vi "test_PhotonPoseEstimator_lowestAmbiguity.vi"(8 "error in (no error)":errorcluster) -> (0 "error out":errorcluster, 3 "Test Passed":bool)   [LabVIEW 2019]
uses:
  <vilib>/Rock Robotics/WPI/ThirdParty/PhotonVisionLib/TypeDef/PhotonEstimatedRobotPoseType.ctl
  <vilib>/Rock Robotics/WPI/ThirdParty/JAS_Junk/TrajLib/TypeDef/POSE3D.ctl
  <vilib>/Rock Robotics/WPI/ThirdParty/JAS_Junk/TrajLib/TypeDef/TRANSLATION3D.ctl
  <vilib>/Rock Robotics/WPI/ThirdParty/JAS_Junk/TrajLib/TypeDef/ROTATION3D.ctl
  <vilib>/Rock Robotics/WPI/ThirdParty/JAS_Junk/TrajLib/TypeDef/QUATERNION.ctl
  <vilib>/Rock Robotics/WPI/ThirdParty/PhotonVisionLib/TypeDef/PhotonTrackedTargetType.ctl
  <vilib>/Rock Robotics/WPI/ThirdParty/PhotonVisionLib/TypeDef/TargetCornerType.ctl
  <vilib>/Rock Robotics/WPI/ThirdParty/JAS_Junk/TrajLib/TypeDef/TRANSFORM3D.ctl
  <vilib>/Rock Robotics/WPI/ThirdParty/PhotonVisionLib/Enum/PhotonPoseStrategy_ENUM.ctl
  <vilib>/Rock Robotics/WPI/ThirdParty/JAS_Junk/TrajLib/VI/Translation3d_Create_Default.vi
  <vilib>/Rock Robotics/WPI/ThirdParty/JAS_Junk/TrajLib/VI/Rotation3d_Create_Default.vi
  <vilib>/Rock Robotics/WPI/ThirdParty/PhotonVisionLib/SubVI/PhotonTargetModel_New_AprilTag36H11.vi
  <vilib>/Rock Robotics/WPI/ThirdParty/JAS_Junk/TrajLib/VI/TimeInterpRotation2d_New.vi
  <vilib>/Rock Robotics/WPI/ThirdParty/JAS_Junk/TrajLib/VI/Quaternion_New.vi
  <vilib>/Rock Robotics/WPI/ThirdParty/PhotonVisionLib/SubVI/PhotonPoseEstimator_Update_All.vi
  <vilib>/Rock Robotics/WPI/ThirdParty/JAS_Junk/TrajLib/VI/Quaternion_New_Default.vi
  <vilib>/Rock Robotics/WPI/ThirdParty/PhotonVisionLib/SubVI/PhotonTargetModel_New_RectPlanar.vi
  <vilib>/Rock Robotics/WPI/ThirdParty/JAS_Junk/TrajLib/Conv_Inches_Meters.vi
  <vilib>/Rock Robotics/WPI/ThirdParty/PhotonVisionLib/SubVI/PhotonPoseEstimator_SetLastPose.vi
  <vilib>/Rock Robotics/WPI/ThirdParty/PhotonVisionLib/SubVI/PhotonPoseEstimator_GetEmptyPose.vi
  <vilib>/Rock Robotics/WPI/ThirdParty/PhotonVisionLib/SubVI/PhotonPoseEstimator_EstimateLowestAmbiguityPose.vi
  <vilib>/Rock Robotics/WPI/ThirdParty/PhotonVisionLib/SubVI/PhotonPoseEstimator_EstimateClosestToCameraHeightPose.vi
  <vilib>/Rock Robotics/WPI/ThirdParty/PhotonVisionLib/SubVI/PhotonPoseEstimator_EstimateClosestToReferencePose.vi
  <vilib>/Rock Robotics/WPI/ThirdParty/PhotonVisionLib/SubVI/PhotonPoseEstimator_GetReferencePose.vi
  <vilib>/Rock Robotics/WPI/ThirdParty/PhotonVisionLib/SubVI/PhotonPoseEstimator_GetLastPose.vi
  <vilib>/Rock Robotics/WPI/ThirdParty/PhotonVisionLib/SubVI/PhotonPoseEstimator_SetReferencePose.vi
  <vilib>/Rock Robotics/WPI/ThirdParty/PhotonVisionLib/SubVI/PhotonPoseEstimator_EstimateClosestToLastPose.vi
  <vilib>/Rock Robotics/WPI/ThirdParty/PhotonVisionLib/SubVI/PhotonPoseEstimator_EstimateAverageBestTargetsPose.vi
  <vilib>/Rock Robotics/WPI/ThirdParty/PhotonVisionLib/SubVI/PhotonPoseEstimator_EstimateMultiTagOnCoprocPose.vi
  <vilib>/Rock Robotics/WPI/ThirdParty/PhotonVisionLib/SubVI/PhotonPoseEstimator_EstimatePnpDistanceTrigSolvePose.vi
  <vilib>/Rock Robotics/WPI/ThirdParty/PhotonVisionLib/SubVI/PhotonPoseEstimator_Strategy_constrainedPnpStrategy.vi
  <vilib>/Rock Robotics/WPI/ThirdParty/PhotonVisionLib/SubVI/PhotonPipelineResult_GetTimeStampSecs.vi
  <vilib>/Rock Robotics/WPI/ThirdParty/PhotonVisionLib/SubVI/PhotonTargetModel_New.vi
  <vilib>/Rock Robotics/WPI/ThirdParty/JAS_Junk/TrajLib/VI/Rotation3d_Create_AxisAngle.vi
  <vilib>/Rock Robotics/WPI/ThirdParty/JAS_Junk/TrajLib/VI/Pose3d_New.vi
  <vilib>/Rock Robotics/WPI/ThirdParty/PhotonVisionLib/SubVI/PhotonPipelineResult_HasTargets.vi
  <vilib>/Rock Robotics/WPI/ThirdParty/PhotonVisionLib/SubVI/PhotonPipelineResult_GetTargets.vi
  <vilib>/Rock Robotics/WPI/ThirdParty/PhotonVisionLib/SubVI/PhotonTrackedTarget_GetPoseAmbiguity.vi
  <vilib>/Rock Robotics/WPI/ThirdParty/PhotonVisionLib/SubVI/PhotonTrackedTarget_GetFiducialId.vi
  <vilib>/Rock Robotics/WPI/ThirdParty/PhotonVisionLib/SubVI/PhotonPoseEstimator_GetFieldTags.vi
  <vilib>/Rock Robotics/WPI/ThirdParty/JAS_Junk/TrajLib/VI/AprilTagFieldLayout_GetTagPose.vi
  <vilib>/Rock Robotics/WPI/ThirdParty/JAS_Junk/TrajLib/VI/Pose3d_TransformBy.vi
  <vilib>/Rock Robotics/WPI/ThirdParty/PhotonVisionLib/SubVI/PhotonTrackedTarget_GetBestCameraToTarget.vi
  <vilib>/Rock Robotics/WPI/ThirdParty/JAS_Junk/TrajLib/VI/Transform3d_Inverse.vi
  <vilib>/Rock Robotics/WPI/ThirdParty/PhotonVisionLib/SubVI/PhotonPoseEstimator_GetRobotToCameraTransform.vi
  <vilib>/Rock Robotics/WPI/ThirdParty/PhotonVisionLib/SubVI/PhotonPoseEstimator_GetHighestAmbiguity.vi
  <vilib>/Rock Robotics/WPI/ThirdParty/PhotonVisionLib/SubVI/PhotonEstimatedRobotPose_New.vi
  <vilib>/Rock Robotics/WPI/ThirdParty/PhotonVisionLib/SubVI/PhotonPoseEstimator_Strategy_closestToCameraHeight_calc.vi
  <vilib>/Rock Robotics/WPI/ThirdParty/PhotonVisionLib/SubVI/PhotonTrackedTarget_GetAltCameraToTarget.vi
  <vilib>/Rock Robotics/WPI/ThirdParty/PhotonVisionLib/SubVI/PhotonPoseEstimator_Strategy_closestToReferencePose_calc.vi
  <vilib>/Rock Robotics/WPI/ThirdParty/PhotonVisionLib/SubVI/PhotonPoseEstimator_Strategy_averageBestTargets_calc.vi
  <vilib>/Rock Robotics/WPI/ThirdParty/JAS_Junk/TrajLib/VI/Rotation3d_Plus.vi
  <vilib>/Rock Robotics/WPI/ThirdParty/JAS_Junk/TrajLib/VI/Translation3d_Plus.vi
  <vilib>/Rock Robotics/WPI/ThirdParty/JAS_Junk/TrajLib/VI/Translation3d_Times.vi
  <vilib>/Rock Robotics/WPI/ThirdParty/JAS_Junk/TrajLib/VI/Rotation3d_Times.vi
  <vilib>/Rock Robotics/WPI/ThirdParty/JAS_Junk/TrajLib/VI/Pose3d_New_Trans3dRot3d.vi
  <vilib>/Rock Robotics/WPI/ThirdParty/JAS_Junk/TrajLib/VI/Pose3d_New_Default.vi
  <vilib>/Rock Robotics/WPI/ThirdParty/JAS_Junk/TrajLib/VI/Pose3d_Plus.vi
  <vilib>/Rock Robotics/WPI/ThirdParty/JAS_Junk/TrajLib/VI/Pose3d_RelativeTo.vi
  <vilib>/Rock Robotics/WPI/ThirdParty/JAS_Junk/TrajLib/VI/AprilTagFieldLayout_GetOriginPosition.vi
  <vilib>/Rock Robotics/WPI/ThirdParty/PhotonVisionLib/SubVI/PhotonPipelineResult_GetMultiTagResult.vi
  <vilib>/Rock Robotics/WPI/ThirdParty/PhotonVisionLib/SubVI/PhotonPipelineResult_GetBestTarget.vi
  <vilib>/Rock Robotics/WPI/ThirdParty/PhotonVisionLib/SubVI/PhotonTrackedTarget_GetPitch.vi
  <vilib>/Rock Robotics/WPI/ThirdParty/PhotonVisionLib/SubVI/PhotonTrackedTarget_GetYaw.vi
  <vilib>/Rock Robotics/WPI/ThirdParty/JAS_Junk/TrajLib/Units_DegreesToRadians.vi
  <vilib>/Rock Robotics/WPI/ThirdParty/JAS_Junk/TrajLib/VI/Transform3d_GetTranslation3d.vi
  <vilib>/Rock Robotics/WPI/ThirdParty/JAS_Junk/TrajLib/VI/Translation3d_GetNorm.vi
  <vilib>/Rock Robotics/WPI/ThirdParty/JAS_Junk/TrajLib/VI/Translation3d_Create_DistAng.vi
  <vilib>/Rock Robotics/WPI/ThirdParty/JAS_Junk/TrajLib/VI/Translation3d_RotateBy.vi
  <vilib>/Rock Robotics/WPI/ThirdParty/JAS_Junk/TrajLib/VI/Translation3d_ToTranslation2d.vi
  <vilib>/Rock Robotics/WPI/ThirdParty/JAS_Junk/TrajLib/Translation2d_RotateBy.vi
  <vilib>/Rock Robotics/WPI/ThirdParty/JAS_Junk/TrajLib/VI/Transform3d_GetRotation3d.vi
  <vilib>/Rock Robotics/WPI/ThirdParty/JAS_Junk/TrajLib/VI/Pose3d_ToPose2d.vi
  <vilib>/Rock Robotics/WPI/ThirdParty/JAS_Junk/TrajLib/Pose2d_getTranslation.vi
  <vilib>/Rock Robotics/WPI/ThirdParty/JAS_Junk/TrajLib/Translation2d_Plus.vi
  <vilib>/Rock Robotics/WPI/ThirdParty/JAS_Junk/TrajLib/Translation2d_UnaryMinus.vi
  <vilib>/Rock Robotics/WPI/ThirdParty/JAS_Junk/TrajLib/Pose2d_New_TRRO.vi
  <vilib>/Rock Robotics/WPI/ThirdParty/JAS_Junk/TrajLib/VI/Pose3d_New_Pose2d.vi
  <vilib>/Rock Robotics/WPI/ThirdParty/JAS_Junk/TrajLib/VI/TimeInterpRotation2d_GetSample.vi
  <vilib>/Rock Robotics/WPI/ThirdParty/PhotonVisionLib/SubVI/PhotonPoseEstimator_GetHeadingBuffer.vi
  <vilib>/Rock Robotics/WPI/ThirdParty/JAS_Junk/TrajLib/VI/Vector_Norm.vi
  <vilib>/Rock Robotics/WPI/ThirdParty/JAS_Junk/TrajLib/VecBuilder_ArrayBy1Fill.vi
  <vilib>/Rock Robotics/WPI/ThirdParty/JAS_Junk/TrajLib/VI/AprilTag_GetAll.vi
  <vilib>/Rock Robotics/WPI/ThirdParty/JAS_Junk/TrajLib/VI/Pose3d_getTranslation3d.vi
  <vilib>/Rock Robotics/WPI/ThirdParty/JAS_Junk/TrajLib/VI/Pose3d_getRotation3d.vi
  <vilib>/Rock Robotics/WPI/ThirdParty/JAS_Junk/TrajLib/VI/Rotation3d_ToRotation2d.vi
  <vilib>/Rock Robotics/WPI/ThirdParty/JAS_Junk/TrajLib/Transform2d_Create_TransRot.vi
  <vilib>/Rock Robotics/WPI/ThirdParty/JAS_Junk/TrajLib/VI/Rotation3d_UnaryMinus.vi
  <vilib>/Rock Robotics/WPI/ThirdParty/JAS_Junk/TrajLib/VI/Translation3d_UnaryMinus.vi
  <vilib>/Rock Robotics/WPI/ThirdParty/JAS_Junk/TrajLib/VI/Transform3d_GetXYZ.vi
  <vilib>/Rock Robotics/WPI/ThirdParty/JAS_Junk/TrajLib/VI/Pose3d_getXYZ.vi
  <vilib>/Rock Robotics/WPI/ThirdParty/PhotonVisionLib/SubVI/PhotonPoseEstimator_CalcDifference.vi
  <vilib>/Rock Robotics/WPI/ThirdParty/JAS_Junk/TrajLib/VI/Rotation3d_RotateBy.vi
  <vilib>/Rock Robotics/WPI/ThirdParty/JAS_Junk/TrajLib/VI/Translation3d_GetXYZ.vi
  <vilib>/Rock Robotics/WPI/ThirdParty/JAS_Junk/TrajLib/VI/Rotation3d_GetQuaterion.vi
  <vilib>/Rock Robotics/WPI/ThirdParty/JAS_Junk/TrajLib/VI/Quaternion_Get_Vect.vi
  <vilib>/Rock Robotics/WPI/ThirdParty/JAS_Junk/TrajLib/VI/Quaternion_Get_W.vi
  <vilib>/Rock Robotics/WPI/ThirdParty/JAS_Junk/TrajLib/VI/Transform3d_Create_Pose3dPose3d.vi
  <vilib>/Rock Robotics/WPI/ThirdParty/JAS_Junk/TrajLib/Conv_Deg_Radians.vi
  <vilib>/Rock Robotics/WPI/ThirdParty/JAS_Junk/TrajLib/VI/Quaternion_Times.vi
  <vilib>/Rock Robotics/WPI/ThirdParty/JAS_Junk/TrajLib/VI/Quaternion_Inverse.vi
  <vilib>/Rock Robotics/WPI/ThirdParty/JAS_Junk/TrajLib/VI/Quaternion_Get_All.vi
  <vilib>/Rock Robotics/WPI/ThirdParty/JAS_Junk/TrajLib/Translation2d_Create.vi
  <vilib>/Rock Robotics/WPI/ThirdParty/JAS_Junk/TrajLib/Pose2d_getXYAngle.vi
  <vilib>/Rock Robotics/WPI/ThirdParty/JAS_Junk/TrajLib/Rotation2d_Interpolate.vi
  <vilib>/Rock Robotics/WPI/ThirdParty/JAS_Junk/TrajLib/MatBuilder_Create.vi
  <vilib>/Rock Robotics/WPI/ThirdParty/JAS_Junk/TrajLib/Rotation2d_CreateAngle.vi
  <vilib>/Rock Robotics/WPI/ThirdParty/JAS_Junk/TrajLib/VI/Rotation3d_GetXYZ.vi
  <vilib>/Rock Robotics/WPI/ThirdParty/JAS_Junk/TrajLib/VI/Rotation3d_Create_Quaternion.vi
  <vilib>/Rock Robotics/WPI/ThirdParty/JAS_Junk/TrajLib/VI/Translation3d_GetDistance.vi
  <vilib>/Rock Robotics/WPI/ThirdParty/JAS_Junk/TrajLib/VI/Translation3d_Minus.vi
  <vilib>/Rock Robotics/WPI/ThirdParty/JAS_Junk/TrajLib/VI/Rotation3d_Minus.vi
  <vilib>/Rock Robotics/WPI/ThirdParty/JAS_Junk/TrajLib/Rotation2d_Plus.vi
  <vilib>/Rock Robotics/WPI/ThirdParty/JAS_Junk/TrajLib/Rotation2d_Minus.vi
  <vilib>/Rock Robotics/WPI/ThirdParty/JAS_Junk/TrajLib/MathUtil_Clamp.vi
  <vilib>/Rock Robotics/WPI/ThirdParty/JAS_Junk/TrajLib/Rotation2d_Times.vi
  <vilib>/Rock Robotics/WPI/ThirdParty/JAS_Junk/TrajLib/VI/Quaternion_Normalize.vi
  <vilib>/Rock Robotics/WPI/ThirdParty/JAS_Junk/TrajLib/Rotation2d_RotateBy.vi
  <vilib>/Rock Robotics/WPI/ThirdParty/JAS_Junk/TrajLib/Rotation2d_UnaryMinus.vi
  <vilib>/Rock Robotics/WPI/ThirdParty/JAS_Junk/TrajLib/Rotation2d_CreateXY.vi
  <vilib>/Rock Robotics/WPI/ThirdParty/JAS_Junk/TrajLib/Util_CalcDist.vi
  <vilib>/Rock Robotics/WPI/ThirdParty/PhotonVisionLib/SubVI/PhotonVision_Globals.vi
  <vilib>/gmath/interp.llb/Search Ordered Table.vi
  <vilib>/Rock Robotics/WPI/ThirdParty/JAS_Junk/TrajLib/Trajectory_Library.lvlib
  <vilib>/Rock Robotics/WPI/ThirdParty/PhotonVisionLib/PhotonVisionLib.lvlib
panel:
  out "Test 2 Passed":bool
  out "Test 1 Passed":bool
  out "Pos Found":bool
  out "PhotonEstimatedRobotPose":T1={"EstimatedPose"={"Translation3d"={"X"=0.0, "Y"=0.0, "Z"=0.0}, "Rotation3d"={"Q_quaternion"={"R"=1.0, "V"=[0.0, 0.0, 0.0]}}}, "TimeStamp_Seconds"=0.0, "targetsUsed"=[], "Strategy"=enum."LOWEST_AMBIGUITY"} {"targetsUsed"."AltCameraToTarget"."TRANSLATION3D"."Z" format="%14.3f"; "targetsUsed"."AltCameraToTarget"."TRANSLATION3D"."Y" format="%14.3f"; "targetsUsed"."AltCameraToTarget"."TRANSLATION3D"."X" format="%14.3f"; "targetsUsed"."BestCameraToTarget"."TRANSLATION3D"."Z" format="%14.3f"; "targetsUsed"."BestCameraToTarget"."TRANSLATION3D"."Y" format="%14.3f"; "targetsUsed"."BestCameraToTarget"."TRANSLATION3D"."X" format="%14.3f"; "EstimatedPose"."Translation3d"."Z" format="%14.3f"; "EstimatedPose"."Translation3d"."Y" format="%14.3f"; "EstimatedPose"."Translation3d"."X" format="%14.3f"}
  out "Test 0 Passed":bool
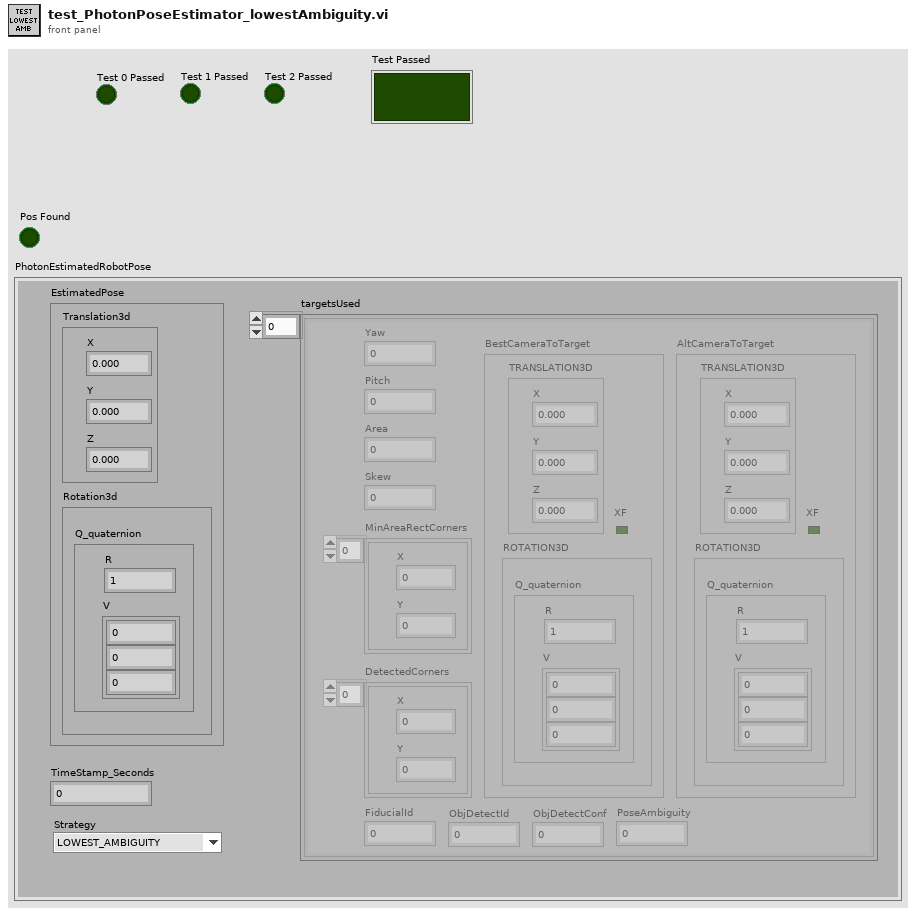
[diagram p1: front panel]
types:
  T1 = typedef "PhotonVisionLib.lvlib/PhotonEstimatedRobotPoseType.ctl" = cluster{"EstimatedPose":T2, "TimeStamp_Seconds":dbl, "targetsUsed":T6[], "Strategy":T9}
  T2 = typedef "Trajectory_Library.lvlib/POSE3D.ctl" = cluster{"Translation3d":T3, "Rotation3d":T4}
  T3 = typedef "Trajectory_Library.lvlib/TRANSLATION3D.ctl" = cluster{"X":dbl, "Y":dbl, "Z":dbl}
  T4 = typedef "Trajectory_Library.lvlib/ROTATION3D.ctl" = cluster{"Q_quaternion":T5}
  T5 = typedef "Trajectory_Library.lvlib/QUATERNION.ctl" = cluster{"R":dbl, "V":dbl[]}
  T6 = typedef "PhotonVisionLib.lvlib/PhotonTrackedTargetType.ctl" = cluster{"Yaw":dbl, "Pitch":dbl, "Area":dbl, "Skew":dbl, "MinAreaRectCorners":T7[], "BestCameraToTarget":T8, "FiducialId":i32, "AltCameraToTarget":T8, "PoseAmbiguity":dbl, "DetectedCorners":T7[], "ObjDetectId":i32, "ObjDetectConf":sgl}
  T7 = typedef "PhotonVisionLib.lvlib/TargetCornerType.ctl" = cluster{"X":dbl, "Y":dbl}
  T8 = typedef "Trajectory_Library.lvlib/TRANSFORM3D.ctl" = cluster{"TRANSLATION3D":T3, "ROTATION3D":T4, "XF":bool}
  T9 = typedef "PhotonVisionLib.lvlib/PhotonPoseStrategy_ENUM.ctl" = enum16{"LOWEST_AMBIGUITY", "CLOSEST_TO_CAMERA_HEIGHT", "CLOSEST_TO_REFERENCE_POSE", "CLOSEST_TO_LAST_POSE", "AVERAGE_BEST_TARGETS", "MULTI_TAG_PNP_ON_COPROCESSOR", "MULTI_TAG_PNP_ON_RIO", "PNP_DISTANCE_TRIG_SOLVE", "CONSTRAINED_SOLVEPNP"}
  T10 = typedef "Trajectory_Library.lvlib/AprilTagFieldLayout.ctl" = cluster{"AprilTagMap":map{i32, T11}, "FieldLength":dbl, "FieldWidth":dbl, "OriginPosition ":T12, "OriginPose3d":T2}
  T11 = typedef "Trajectory_Library.lvlib/AprilTag.ctl" = cluster{"ID":i32, "POSE3D":T2}
  T12 = typedef "Trajectory_Library.lvlib/AprilTagFieldLayoutOrignPosition_ENUM.ctl" = enum16{"kBlueAllianceWallRightSide,", "kRedAllianceWallRightSide,"}
  T13 = typedef "PhotonVisionLib.lvlib/PhotonPipelineMetadataType.ctl" = cluster{"CaptureTimestampMicros":i64, "PublishTimestampMicros":i64, "SequenceID":i64, "TimeSinceLastPong":i64}
  T14 = typedef "PhotonVisionLib.lvlib/PhotonPipelineResultType.ctl" = cluster{"Targets":T6[], "PhotonMultiTargetPNPResult":T15, "PhotonPipelineMetadata":T13}
  T15 = typedef "PhotonVisionLib.lvlib/PhotonMultiTargetPNPResultType.ctl" = cluster{"PhotonPNPResult":T16, "FiducialIDsUsed":i16[]}
  T16 = typedef "PhotonVisionLib.lvlib/PhotonPNPResultType.ctl" = cluster{"IsPresent":bool, "bestReprojErr":dbl, "altReprojErr":dbl, "ambiguity":dbl, "Best":T8, "Alt":T8}
  T17 = typedef "PhotonVisionLib.lvlib/PhotonPoseEstimatorType.ctl" = cluster{"LastPose":T2, "ReferencePose":T2, "FieldTags":T10, "PrimaryStratety":T9, "Camera":string, "RobotToCamera":T8, "ReportedErrors":dbl[], "HighestAmbiguity":dbl, "MultiTagFallbackStrategy":T9, "PoseCacheTimeoutSec":dbl, "PhotonTargetModel":T18, "BaseNTName":string}
  T18 = typedef "PhotonVisionLib.lvlib/PhotonTargetModel.ctl" = cluster{"Vertices":T3[], "IsPlaner":bool, "IsSpherical":bool}
  T19 = typedef "PhotonVisionLib.lvlib/PhotonPoseEstimator_Configuration.ctl" = cluster{"Primary Strategy":T9, "Camera":string, "Initial Pose":T2, "HighestAmbiguity":dbl, "RobotToCamera":T8, "FallBack Strategy":T9, "BaseNTName":string}
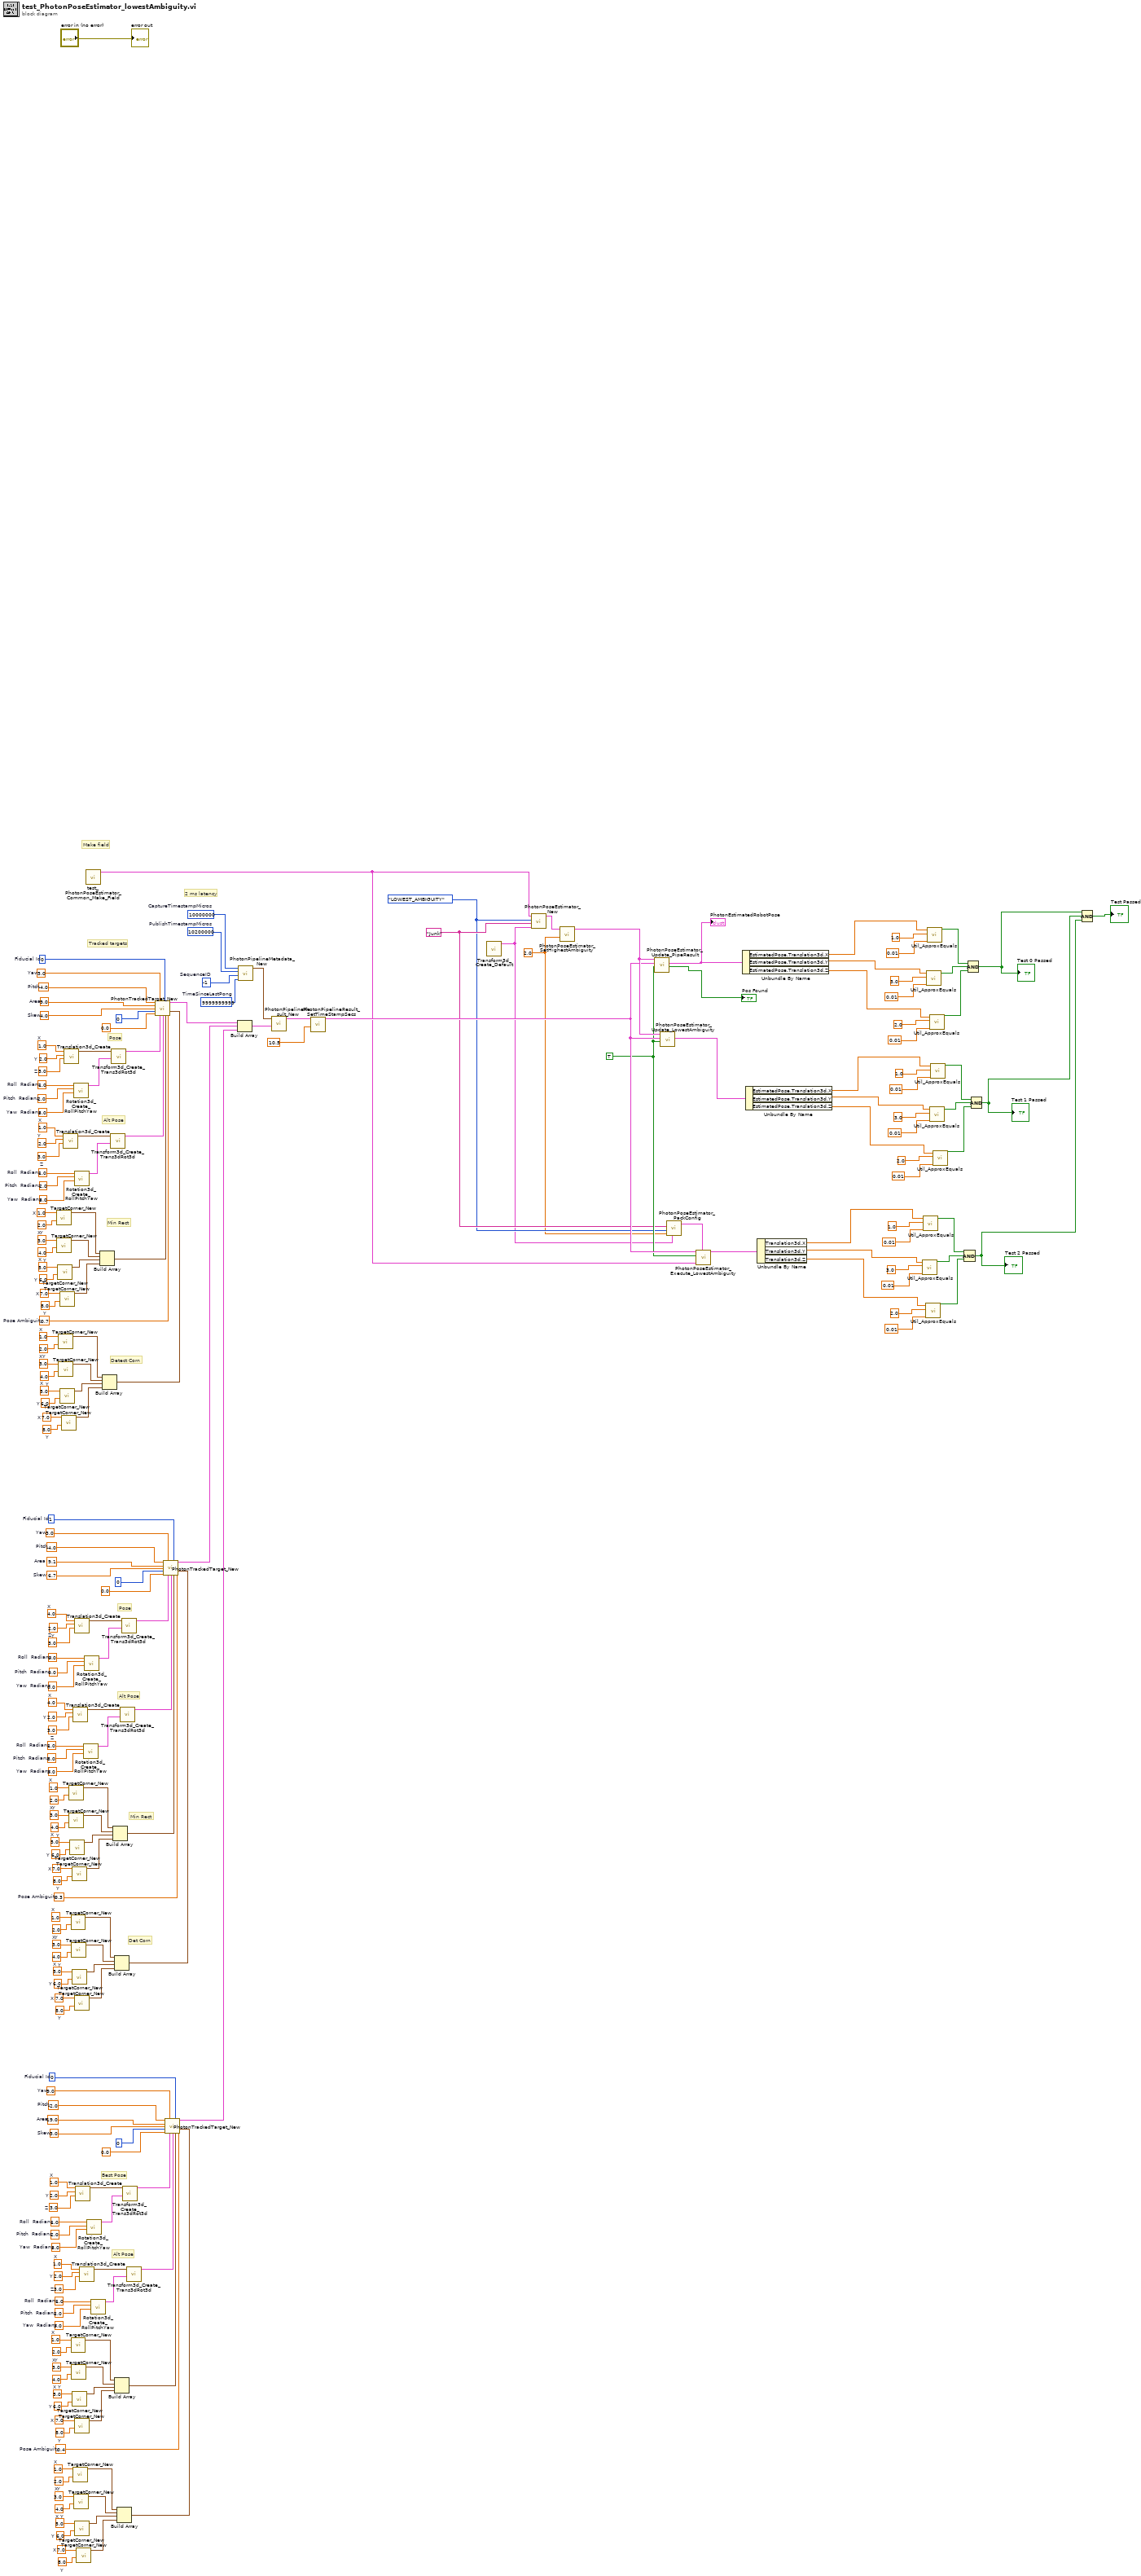
[diagram p0: block diagram]
diagram:
  w2 = 2.0 ("HighestAmbiguity")
  w46 = i64 10000000  # CaptureTimestampMicros
  w47 = i64 10200000  # PublishTimestampMicros
  w48 = i64 -1  # SequenceID
  w49 = i64 9999999999  # TimeSinceLastPong
  w20 = TRUE ("Has Results")
  w4 = "Junk" ("Camera")
  w3 = PhotonPoseStrategy_ENUM."LOWEST_AMBIGUITY" ("Strategy")
  w73 = 1.0  # Roll  Radians
  w72 = 2.0  # Pitch  Radians
  w71 = 3.0  # Yaw  Radians
  w76 = 3.0  # Z
  w75 = 1.0  # X
  w74 = 2.0  # Y
  w81 = 1.0  # Roll  Radians
  w80 = 2.0  # Pitch  Radians
  w79 = 3.0  # Yaw  Radians
  w84 = 3.0  # Z
  w83 = 1.0  # X
  w82 = 2.0  # Y
  w91 = 7.0  # X
  w92 = 8.0  # Y
  w93 = 5.0  # X
  w94 = 6.0  # Y
  w95 = 3.0  # X
  w96 = 4.0  # Y
  w97 = 1.0  # X
  w98 = 2.0  # Y
  w103 = 7.0  # X
  w104 = 8.0  # Y
  w105 = 5.0  # X
  w106 = 6.0  # Y
  w107 = 3.0  # X
  w108 = 4.0  # Y
  w109 = 1.0  # X
  w110 = 2.0  # Y
  w111 = -2.0  # Pitch
  w112 = 19.0  # Area
  w113 = 3.0  # Skew
  w114 = 0  # Fiducial Id
  w115 = 0.4  # Pose Ambiguity
  w116 = 9.0  # Yaw
  w123 = 0.0  # Roll  Radians
  w122 = 0.0  # Pitch  Radians
  w121 = 0.0  # Yaw  Radians
  w126 = 3.0  # Z
  w125 = 4.0  # X
  w124 = 2.0  # Y
  w131 = 1.0  # Roll  Radians
  w130 = 5.0  # Pitch  Radians
  w129 = 3.0  # Yaw  Radians
  w134 = 3.0  # Z
  w133 = 4.0  # X
  w132 = 2.0  # Y
  w141 = 7.0  # X
  w142 = 8.0  # Y
  w143 = 5.0  # X
  w144 = 6.0  # Y
  w145 = 3.0  # X
  w146 = 4.0  # Y
  w147 = 1.0  # X
  w148 = 2.0  # Y
  w153 = 7.0  # X
  w154 = 8.0  # Y
  w155 = 5.0  # X
  w156 = 6.0  # Y
  w157 = 3.0  # X
  w158 = 4.0  # Y
  w159 = 1.0  # X
  w160 = 2.0  # Y
  w161 = -4.0  # Pitch
  w162 = 9.1  # Area
  w163 = 6.7  # Skew
  w164 = 1  # Fiducial Id
  w165 = 0.3  # Pose Ambiguity
  w166 = 3.0  # Yaw
  w173 = 1.0  # Roll  Radians
  w172 = 2.0  # Pitch  Radians
  w171 = 3.0  # Yaw  Radians
  w176 = 3.0  # Z
  w175 = 1.0  # X
  w174 = 2.0  # Y
  w181 = 1.0  # Roll  Radians
  w180 = 2.0  # Pitch  Radians
  w179 = 3.0  # Yaw  Radians
  w184 = 3.0  # Z
  w183 = 1.0  # X
  w182 = 2.0  # Y
  w191 = 7.0  # X
  w192 = 8.0  # Y
  w193 = 5.0  # X
  w194 = 6.0  # Y
  w195 = 3.0  # X
  w196 = 4.0  # Y
  w197 = 1.0  # X
  w198 = 2.0  # Y
  w203 = 7.0  # X
  w204 = 8.0  # Y
  w205 = 5.0  # X
  w206 = 6.0  # Y
  w207 = 3.0  # X
  w208 = 4.0  # Y
  w209 = 1.0  # X
  w210 = 2.0  # Y
  w211 = -4.0  # Pitch
  w212 = 9.0  # Area
  w213 = 4.0  # Skew
  w214 = 0  # Fiducial Id
  w215 = 0.7  # Pose Ambiguity
  w216 = 3.0  # Yaw
  # "2 ms latency"
  # "Det Corn"
  # "Min Rect"
  # "Pose"
  # "Detect Corn"
  # "Min Rect"
  # "Tracked targets"
  # "Make field"
  # "Best Pose"
  # "Alt Pose"
  # "Alt Pose"
  # "Pose"
  # "Alt Pose"
  n1 = call <vilib>:"TargetCorner_New.vi"("Y"=w210, "X"=w209) -> ("TargetCorner"=w202:T7)  [unwired: 9 in]
  n2 = call <vilib>:"TargetCorner_New.vi"("Y"=w208, "X"=w207) -> ("TargetCorner"=w201:T7)  [unwired: 9 in]
  n3 = call <vilib>:"TargetCorner_New.vi"("Y"=w206, "X"=w205) -> ("TargetCorner"=w200:T7)  [unwired: 9 in]
  n4 = call <vilib>:"TargetCorner_New.vi"("Y"=w198, "X"=w197) -> ("TargetCorner"=w190:T7)  [unwired: 9 in]
  n5 = call <vilib>:"TargetCorner_New.vi"("Y"=w196, "X"=w195) -> ("TargetCorner"=w189:T7)  [unwired: 9 in]
  n6 = call <vilib>:"TargetCorner_New.vi"("Y"=w204, "X"=w203) -> ("TargetCorner"=w199:T7)  [unwired: 9 in]
  n7 = call <vilib>:"TargetCorner_New.vi"("Y"=w194, "X"=w193) -> ("TargetCorner"=w188:T7)  [unwired: 9 in]
  n8 = call <vilib>:"TargetCorner_New.vi"("Y"=w192, "X"=w191) -> ("TargetCorner"=w187:T7)  [unwired: 9 in]
  n9 = call <vilib>:"Translation3d_Create.vi"("Z"=w184, "Y"=w182, "X"=w183) -> ("TRANSLATION3D"=w178:T3)  [unwired: 8 in]
  n10 = call <vilib>:"Translation3d_Create.vi"("Z"=w176, "Y"=w174, "X"=w175) -> ("TRANSLATION3D"=w170:T3)  [unwired: 8 in]
  n11 = call <vilib>:"TargetCorner_New.vi"("Y"=w160, "X"=w159) -> ("TargetCorner"=w152:T7)  [unwired: 9 in]
  n12 = call <vilib>:"TargetCorner_New.vi"("Y"=w158, "X"=w157) -> ("TargetCorner"=w151:T7)  [unwired: 9 in]
  n13 = call <vilib>:"TargetCorner_New.vi"("Y"=w156, "X"=w155) -> ("TargetCorner"=w150:T7)  [unwired: 9 in]
  n14 = call <vilib>:"TargetCorner_New.vi"("Y"=w148, "X"=w147) -> ("TargetCorner"=w140:T7)  [unwired: 9 in]
  n15 = call <vilib>:"TargetCorner_New.vi"("Y"=w110, "X"=w109) -> ("TargetCorner"=w102:T7)  [unwired: 9 in]
  n16 = call <vilib>:"TargetCorner_New.vi"("Y"=w146, "X"=w145) -> ("TargetCorner"=w139:T7)  [unwired: 9 in]
  n17 = call <vilib>:"TargetCorner_New.vi"("Y"=w108, "X"=w107) -> ("TargetCorner"=w101:T7)  [unwired: 9 in]
  n18 = call <vilib>:"TargetCorner_New.vi"("Y"=w154, "X"=w153) -> ("TargetCorner"=w149:T7)  [unwired: 9 in]
  n19 = call <vilib>:"TargetCorner_New.vi"("Y"=w144, "X"=w143) -> ("TargetCorner"=w138:T7)  [unwired: 9 in]
  n20 = call <vilib>:"TargetCorner_New.vi"("Y"=w106, "X"=w105) -> ("TargetCorner"=w100:T7)  [unwired: 9 in]
  n21 = call <vilib>:"Translation3d_Create.vi"("Z"=w134, "Y"=w132, "X"=w133) -> ("TRANSLATION3D"=w128:T3)  [unwired: 8 in]
  n22 = call <vilib>:"TargetCorner_New.vi"("Y"=w98, "X"=w97) -> ("TargetCorner"=w90:T7)  [unwired: 9 in]
  n23 = call <vilib>:"Rotation3d_Create_RollPitchYaw.vi"("Yaw"=w171, "Pitch"=w172, "Roll"=w173) -> ("Rotation3d"=w169:T4)  [unwired: 8 in]
  n24 = call <vilib>:"TargetCorner_New.vi"("Y"=w96, "X"=w95) -> ("TargetCorner"=w89:T7)  [unwired: 9 in]
  n25 = call <vilib>:"Rotation3d_Create_RollPitchYaw.vi"("Yaw"=w179, "Pitch"=w180, "Roll"=w181) -> ("Rotation3d"=w177:T4)  [unwired: 8 in]
  n26 = call <vilib>:"Translation3d_Create.vi"("Z"=w126, "Y"=w124, "X"=w125) -> ("TRANSLATION3D"=w120:T3)  [unwired: 8 in]
  n27 = call <vilib>:"TargetCorner_New.vi"("Y"=w142, "X"=w141) -> ("TargetCorner"=w137:T7)  [unwired: 9 in]
  n28 = call <vilib>:"TargetCorner_New.vi"("Y"=w104, "X"=w103) -> ("TargetCorner"=w99:T7)  [unwired: 9 in]
  n29 = call <vilib>:"TargetCorner_New.vi"("Y"=w94, "X"=w93) -> ("TargetCorner"=w88:T7)  [unwired: 9 in]
  n30 = call <vilib>:"Translation3d_Create.vi"("Z"=w76, "Y"=w74, "X"=w75) -> ("TRANSLATION3D"=w70:T3)  [unwired: 8 in]
  n31 = call <vilib>:"TargetCorner_New.vi"("Y"=w92, "X"=w91) -> ("TargetCorner"=w87:T7)  [unwired: 9 in]
  n32 = call <vilib>:"Translation3d_Create.vi"("Z"=w84, "Y"=w82, "X"=w83) -> ("TRANSLATION3D"=w78:T3)  [unwired: 8 in]
  n33 = call <vilib>:"Rotation3d_Create_RollPitchYaw.vi"("Yaw"=w129, "Pitch"=w130, "Roll"=w131) -> ("Rotation3d"=w127:T4)  [unwired: 8 in]
  n34 = call <vilib>:"Rotation3d_Create_RollPitchYaw.vi"("Yaw"=w121, "Pitch"=w122, "Roll"=w123) -> ("Rotation3d"=w119:T4)  [unwired: 8 in]
  n35 = call "test_PhotonPoseEstimator_Common_Make_Field.vi"() -> ("AprilTagFieldLayout"=w19:T10)  [unwired: 11 in]
  n36 = call <vilib>:"Rotation3d_Create_RollPitchYaw.vi"("Yaw"=w71, "Pitch"=w72, "Roll"=w73) -> ("Rotation3d"=w69:T4)  [unwired: 8 in]
  n37 = call <vilib>:"Rotation3d_Create_RollPitchYaw.vi"("Yaw"=w79, "Pitch"=w80, "Roll"=w81) -> ("Rotation3d"=w77:T4)  [unwired: 8 in]
  n38 = Build Array(w202, w201, w200, w199) -> (w186:T7[])
  n39 = Build Array(w190, w189, w188, w187) -> (w185:T7[])
  n40 = call <vilib>:"Transform3d_Create_Trans3dRot3d.vi"("Rotation3d"=w177, "Translation3d"=w178) -> ("Transform3d"=w167:T8)  [unwired: 9 in]
  n41 = call <vilib>:"Transform3d_Create_Trans3dRot3d.vi"("Rotation3d"=w169, "Translation3d"=w170) -> ("Transform3d"=w168:T8)  [unwired: 9 in]
  n42 = Build Array(w152, w151, w150, w149) -> (w136:T7[])
  n43 = Build Array(w140, w139, w138, w137) -> (w135:T7[])
  n44 = Build Array(w102, w101, w100, w99) -> (w86:T7[])
  n45 = Build Array(w90, w89, w88, w87) -> (w85:T7[])
  n46 = call <vilib>:"Transform3d_Create_Trans3dRot3d.vi"("Rotation3d"=w127, "Translation3d"=w128) -> ("Transform3d"=w117:T8)  [unwired: 9 in]
  n47 = call <vilib>:"Transform3d_Create_Trans3dRot3d.vi"("Rotation3d"=w119, "Translation3d"=w120) -> ("Transform3d"=w118:T8)  [unwired: 9 in]
  n48 = call <vilib>:"Transform3d_Create_Trans3dRot3d.vi"("Rotation3d"=w69, "Translation3d"=w70) -> ("Transform3d"=w68:T8)  [unwired: 9 in]
  n49 = call <vilib>:"Transform3d_Create_Trans3dRot3d.vi"("Rotation3d"=w77, "Translation3d"=w78) -> ("Transform3d"=w67:T8)  [unwired: 9 in]
  n50 = call <vilib>:"PhotonTrackedTarget_New.vi"("Pitch"=w211, "Yaw"=w216, "Fiducial Id"=w214, "Area"=w212, "Skew"=w213, "ObjDetectId"=0, "DetectedCorners"=w185, "DetectObjConf"=sgl 0.0, "BestCameraToTarget"=w168, "AltCameraToTarget"=w167, "MinAreaRectCorners"=w186, "Pose Ambiguity"=w215) -> ("TrackedTarget"=w66:T6)  [unwired: 3 in]
  n51 = call <vilib>:"PhotonTrackedTarget_New.vi"("Pitch"=w161, "Yaw"=w166, "Fiducial Id"=w164, "Area"=w162, "Skew"=w163, "ObjDetectId"=0, "DetectedCorners"=w135, "DetectObjConf"=sgl 0.0, "BestCameraToTarget"=w118, "AltCameraToTarget"=w117, "MinAreaRectCorners"=w136, "Pose Ambiguity"=w165) -> ("TrackedTarget"=w65:T6)  [unwired: 3 in]
  n52 = call <vilib>:"PhotonTrackedTarget_New.vi"("Pitch"=w111, "Yaw"=w116, "Fiducial Id"=w114, "Area"=w112, "Skew"=w113, "ObjDetectId"=0, "DetectedCorners"=w85, "DetectObjConf"=sgl 0.0, "BestCameraToTarget"=w68, "AltCameraToTarget"=w67, "MinAreaRectCorners"=w86, "Pose Ambiguity"=w115) -> ("TrackedTarget"=w64:T6)  [unwired: 3 in]
  n53 = Build Array(w66, w65, w64) -> (w63:T6[])
  n54 = call <vilib>:"PhotonPipelineMetadata_New.vi"("TimeSinceLastPong"=w49, "SequenceID"=w48, "PublishTimestampMicros"=w47, "CaptureTimestampMicros"=w46) -> ("PhotonPipelineMetadata"=w45:T13)  [unwired: 7 in]
  n55 = call <vilib>:"PhotonPipelineResult_New.vi"("TrackedTargets"=w63, "Metadata"=w45) -> ("PhotonPipelineResult"=w62:T14)  [unwired: 9 in]
  n56 = call <vilib>:"PhotonPipelineResult_SetTimeStampSecs.vi"("TimeStampSec"=10.5, "PhotonPipelineResult"=w62) -> ("Out PhotonPipelineResult"=w21:T14)  [unwired: 9 in]
  n57 = call <vilib>:"Transform3d_Create_Default.vi"() -> ("Transform3d"=w1:T8)  [unwired: 11 in]
  n58 = call <vilib>:"PhotonPoseEstimator_New.vi"("RobotToCamera"=w1, "Camera"=w4, "Strategy"=w3, "AprilTagFieldLayout"=w19) -> ("PhotonPoseEstimator"=w38:T17)  [unwired: 7 in]
  n59 = call <vilib>:"PhotonPoseEstimator_SetHighestAmbiguity.vi"("HighestAmbiguity"=w2, "PhotonPoseEstimator"=w38) -> ("out PhotonPoseEstimator"=w37:T17)  [unwired: 9 in]
  n60 = call <vilib>:"PhotonPoseEstimator_Update_PipeResult.vi"("Has Results"=w20, "PipelineResult"=w21, "PhotonPoseEstimator"=w37) -> ("Pos Found"=→"Pos Found":bool, "PhotonEstimatedRobotPose"=w51:T1)  [unwired: 6 in, 1 out]
  "PhotonEstimatedRobotPose" <- w51
  n61 = call <vilib>:"PhotonPoseEstimator_Update_LowestAmbiguity.vi"("Has Results"=w20, "PipelineResult"=w21, "PhotonPoseEstimator"=w37) -> ("PhotonEstimatedRobotPose"=w24:T1)  [unwired: 6 in, 2 out]
  n62 = call <vilib>:"PhotonPoseEstimator_PackConfig.vi"("RobotToCamera"=w1, "HighestAmbiguity"=w2, "PirmaryStrategy"=w3, "Camera"=w4) -> ("PoseEstimator_Configuration"=w22:T19)  [unwired: 7 in]
  n63 = call <vilib>:"PhotonPoseEstimator_Execute_LowestAmbiguity.vi"("Configuration"=w22, "AprilTagFieldLayout"=w19, "PIpeline Has \nNew Results"=w20, "PipelineResult"=w21) -> ("EstimatedPose3d"=w6:T2)  [unwired: 2 in, 5 out]
  n64 = Unbundle By Name(w51) -> ("EstimatedPose.Translation3d.X"=w54:dbl, "EstimatedPose.Translation3d.Y"=w53:dbl, "EstimatedPose.Translation3d.Z"=w52:dbl)
  n65 = Unbundle By Name(w24) -> ("EstimatedPose.Translation3d.X"=w27:dbl, "EstimatedPose.Translation3d.Y"=w26:dbl, "EstimatedPose.Translation3d.Z"=w25:dbl)
  n66 = Unbundle By Name(w6) -> ("Translation3d.X"=w9:dbl, "Translation3d.Y"=w8:dbl, "Translation3d.Z"=w7:dbl)
  n67 = call <vilib>:"Util_ApproxEquals.vi"("Tolerance"=0.01, "Value 2"=3.0, "Value 1"=w8) -> ("ApproxEquals"=w11:bool)  [unwired: 8 in]
  n68 = call <vilib>:"Util_ApproxEquals.vi"("Tolerance"=0.01, "Value 2"=1.0, "Value 1"=w9) -> ("ApproxEquals"=w16:bool)  [unwired: 8 in]
  n69 = call <vilib>:"Util_ApproxEquals.vi"("Tolerance"=0.01, "Value 2"=2.0, "Value 1"=w7) -> ("ApproxEquals"=w10:bool)  [unwired: 8 in]
  n70 = call <vilib>:"Util_ApproxEquals.vi"("Tolerance"=0.01, "Value 2"=3.0, "Value 1"=w53) -> ("ApproxEquals"=w56:bool)  [unwired: 8 in]
  n71 = call <vilib>:"Util_ApproxEquals.vi"("Tolerance"=0.01, "Value 2"=1.0, "Value 1"=w54) -> ("ApproxEquals"=w219:bool)  [unwired: 8 in]
  n72 = call <vilib>:"Util_ApproxEquals.vi"("Tolerance"=0.01, "Value 2"=2.0, "Value 1"=w52) -> ("ApproxEquals"=w55:bool)  [unwired: 8 in]
  n73 = call <vilib>:"Util_ApproxEquals.vi"("Tolerance"=0.01, "Value 2"=3.0, "Value 1"=w26) -> ("ApproxEquals"=w29:bool)  [unwired: 8 in]
  n74 = call <vilib>:"Util_ApproxEquals.vi"("Tolerance"=0.01, "Value 2"=1.0, "Value 1"=w27) -> ("ApproxEquals"=w34:bool)  [unwired: 8 in]
  n75 = call <vilib>:"Util_ApproxEquals.vi"("Tolerance"=0.01, "Value 2"=2.0, "Value 1"=w25) -> ("ApproxEquals"=w28:bool)  [unwired: 8 in]
  n76 = Compound Arithmetic op=AND(w16, w11, w10) -> (w5:bool)
  "Test 2 Passed" <- w5
  n77 = Compound Arithmetic op=AND(w219, w56, w55) -> (w217:bool)
  "Test 0 Passed" <- w217
  n78 = Compound Arithmetic op=AND(w34, w29, w28) -> (w23:bool)
  "Test 1 Passed" <- w23
  n79 = Compound Arithmetic op=AND(w217, w23, w5) -> (→"Test Passed":bool)
  "error out" <- "error in (no error)"
